vi "csb frames to pcap range.vi"(0 "n_frames":i32, 1 "first":i32, 2 "max_packets":i32, 3 "t_dev":dbl[](array[numeric]), 4 "id":u32[](array[numeric]), 5 "flags":u16[](array[numeric]), 6 "data_len":u8[](array[numeric]), 7 "error in (no error)":errorcluster, 8 "data":u8[](array[numeric]), 9 "allow":u32[](array[numeric]), 10 "n_allow":i32, 11 "deny":u32[](array[numeric]), 12 "n_deny":i32, 13 "tai_minus_utc_s":i32, 14 "options":i32, 15 "out":u8[](array[numeric]), 16 "out_cap":i32) -> (20 "out out":u8[](array[numeric]), 21 "n_packets":i32, 22 "n_filtered":i32, 23 "n_skipped":i32, 24 "next":i32, 25 "function return":i32, 27 "error out":errorcluster)   [LabVIEW 2021, in "CANsub_Codec.lvlib"]
doc: "int32_t csb_frames_to_pcap_range(int32_t n_frames, int32_t first, int32_t max_packets,\n const double *t_dev, const uint32_t *id, const uint16_t *flags,\n const uint8_t *data_len, const uint8_t *data,\n const uint32_t *allow, int32_t n_allow,\n const uint32_t *deny, int32_t n_deny,\n int32_t tai_minus_utc_s, int32_t options,\n uint8_t *out, int32_t out_cap,\n int32_t *n_packets, int32_t *n_filtered, int32_t *n_skipped, int32_t *next);"
uses:
  CANsub_Codec.lvlib
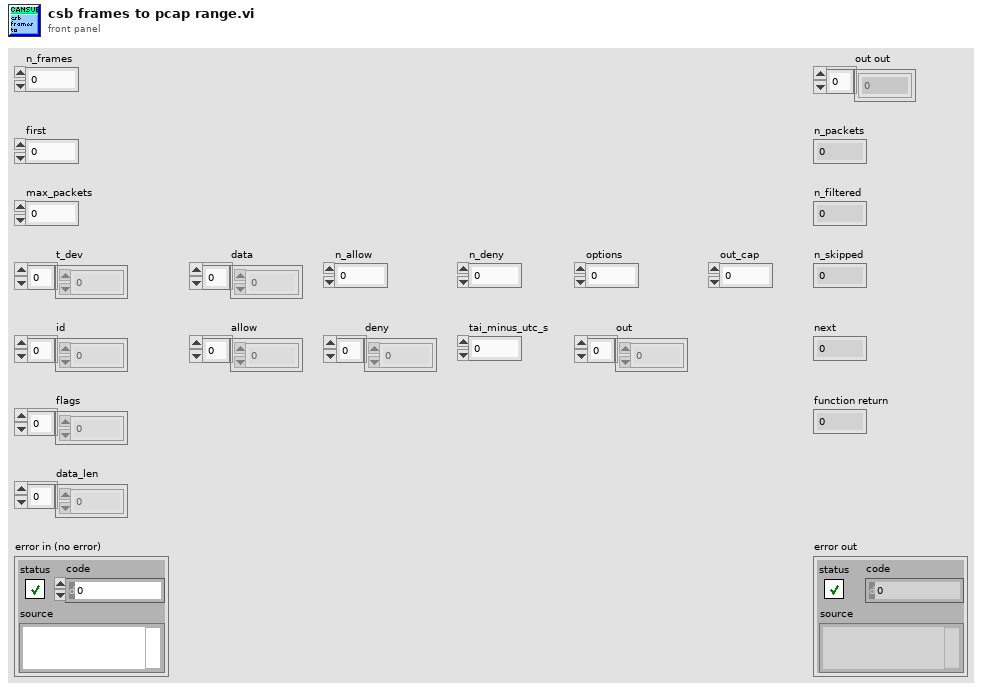
[diagram p1: front panel]
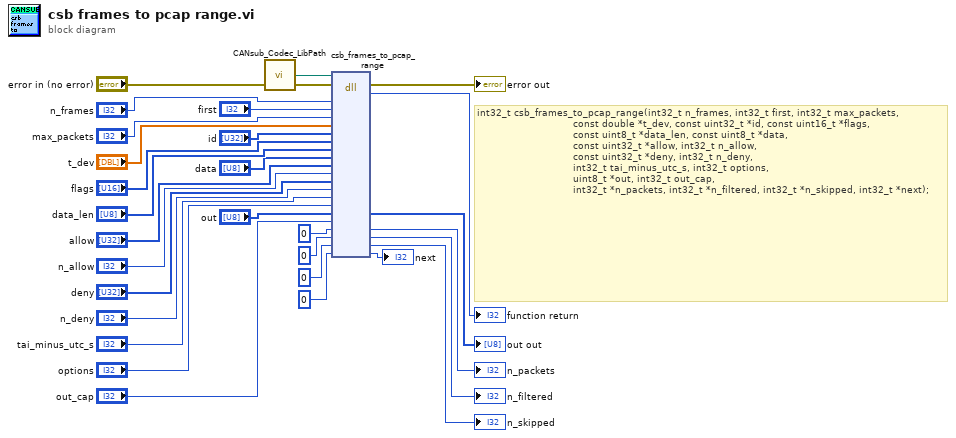
[diagram p0: block diagram]
diagram:
  # "int32_t csb_frames_to_pcap_range(int32_t n_frames, int32_t first, int32_t max_packets,\n                                const double *t_dev, const uint32_t *id, const uint16_t *flags,\n                                const uint8_t *data_len, const uint8_t *data,\n                                const uint32_t *allow, int32_t n_allow,\n                                const uint32_t *deny, int32_t n_deny,\n                                int32_t tai_minus_utc_s, int32_t options,\n                                uint8_t *out, int32_t out_cap,\n                                int32_t *n_packets, int32_t *n_filtered, int32_t *n_skipped, int32_t *next);"
  n1 = call "CANsub_Codec_LibPath.vi"() -> ("Path"=w1:path)  [unwired: 11 in]
  n2 = dll-call lib="libcansub_codec.*" fn="csb_frames_to_pcap_range"(path in=w1, error in="error in (no error)", "n_frames"="n_frames", "first"="first", "max_packets"="max_packets", "t_dev"="t_dev", "id"="id", "flags"="flags", "data_len"="data_len", "data"="data", "allow"="allow", "n_allow"="n_allow", "deny"="deny", "n_deny"="n_deny", "tai_minus_utc_s"="tai_minus_utc_s", "options"="options", "out"="out", "out_cap"="out_cap", "n_packets"=0, "n_filtered"=0, "n_skipped"=0, "next"=0) -> (error out=→"error out":errorcluster, "return type"=→"function return":i32, "out"=→"out out":u8[], "n_packets"=→"n_packets":i32, "n_filtered"=→"n_filtered":i32, "n_skipped"=→"n_skipped":i32, "next"=→"next":i32)  [unwired: 16 in, 1 out]
